vi "Get Size (multiple).vi"(8 "error in (no error)":errorcluster, 11 "XY-data":cluster{"X-array":dbl[], "Y-array":dbl[]}[](array[cluster])) -> (0 "error out":errorcluster, 1 "X size":i32[](array[numeric]), 2 "Y size":i32[](array[numeric]), 3 "XY-data out":cluster{"X-array":dbl[], "Y-array":dbl[]}[](array[cluster]))   [LabVIEW 2019, in "xy_utilities.lvlib"]
doc: "Get size of X and Y arrays."
uses:
  xy_utilities.lvlib
  Get X and Y.vi
  Get X and Y (single).vi
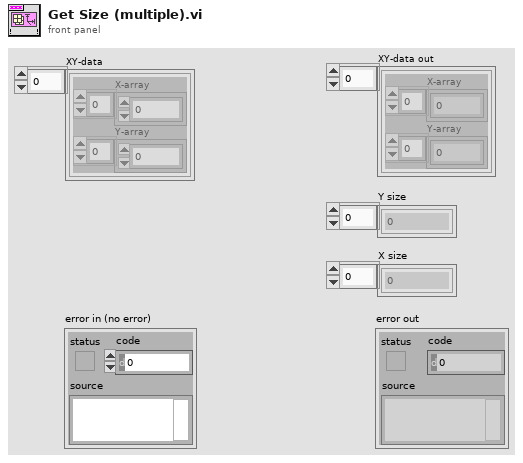
[diagram p1: front panel]
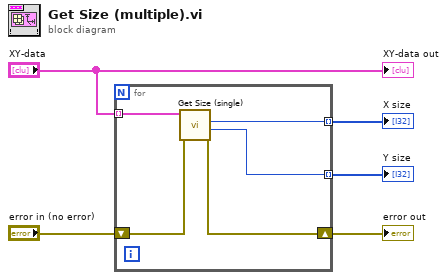
[diagram p0: block diagram]
diagram:
  n1 = for {
    tunnel: "XY-data" -> [w10] mode=indexing
    tunnel: [w9] -> w5 mode=indexing
    tunnel: [w8] -> w4 mode=indexing
    shift-right: [w7] -> w3
    shift-left: "error in (no error)" -> [w6]
    n2 = call "Get Size (single).vi"("error in (no error)"=w6, "XY-data"=w10) -> ("error out"=w7:errorcluster, "X size"=w8:i32, "Y size"=w9:i32)  [unwired: 6 in, 1 out]
  }
  "Y size" <- w4
  "X size" <- w5
  "error out" <- w3
  "XY-data out" <- "XY-data"
